vi "波形图.vi"() -> ()   [LabVIEW 2026]
doc: "波形图界面 - 测控软件 多链路实时波形展示。仅前面板布局演示，无程序逻辑。来源：波形图.html 主界面。"
panel:
  out "运行时长":string="运行时长: 00:00:00"
  out "通道":string="通道: 16"
  out "视图":string="视图: 0.0 - 30.0 s"
  out "窗口":string="窗口: 30.0 s"
  out "采样率":string="采样率: 100 Hz / 10 Hz"
  out "链路":string="链路: 4/4 在线"
  out "?":string="滚轮:缩放时间轴 · 左键框选放大 · 右键平移 · 双击复位"
  out "?":string="Δ值 --"
  out "?":string="Δt --"
  out "?":string="C2 --"
  out "?":string="C1 --"
  out "?":string="测量游标未放置 (0/2)"
  out "?":bool
  out "ARINC429 链路":bool=TRUE
  out "CAN 链路":bool=TRUE
  out "OPC 链路":bool=TRUE
  out "TCP 链路":bool=TRUE
  out "可见通道":i32=16
  out "总通道数":i32=23
  out "绘制帧率":string="60 fps"
  out "重绘周期":string="50 ms"
  out "?":string[](array[string])=["TCP(100 Hz · 10 通道): 转速(rpm) 24800", "TCP: 扭矩(N·m) 745", "TCP: 排气温度(℃) 662", "TCP: 滑油压力(kPa) 348", "TCP: 燃油流量(kg/h) 1240", "TCP: 起动信号 ON", "OPC(10 Hz · 5 通道): 28V母线电压(V) 28.10", "OPC: 28V母线电流(A) 12.40", "CAN(50 Hz · 4 通道): 发电机频率(Hz) 400", "ARINC429(20 Hz · 4 通道): 气压高度(m) 3200", "ARINC429: 马赫数 0.42"]
  out "?":waveform(dbl)(graph)
  out "?":string[](array[string])=["● 下位机 TCP | 192.168.1.101:8000 | PXIE-8840 环形缓冲 | 100 Hz | 10 通道", "● PLC OPC | opc.tcp://192.168.1.50:4840 | 西门子 S7-1500 OPC UA | 10 Hz | 5 通道", "● CAN 总线 | CAN1 · 500 kbps | PCIe-CAN-2 标准帧 | 50 Hz | 4 通道", "● ARINC429 | 429A/L0B1-L0B4 | PXIe-429-4 4发4收 | 20 Hz | 4 通道"]
  in  "通道过滤":i32(ring) items=["全部链路", "仅 TCP", "仅 OPC", "仅 CAN", "仅 ARINC429"]
  in  "Y轴模式":i32(ring) items=["百分比", "物理量程"]
  in  "窗口选择":i32(ring)=30 items=["5 s"=5, "10 s"=10, "15 s"=15, "30 s"=30, "60 s"=60, "120 s"=120]
  in  "清空缓冲":bool
  in  "导出图片":bool
  in  "清除游标":bool
  in  "放置游标":bool
  in  "复位视图":bool
  in  "暂停刷新":bool
  in  "滚动窗口":bool
  out "?":string="--:--:--"
  out "?":string="链路: 4/4 在线"
  out "?":string="● 波形图 | 测控软件 · 多链路实时波形展示"
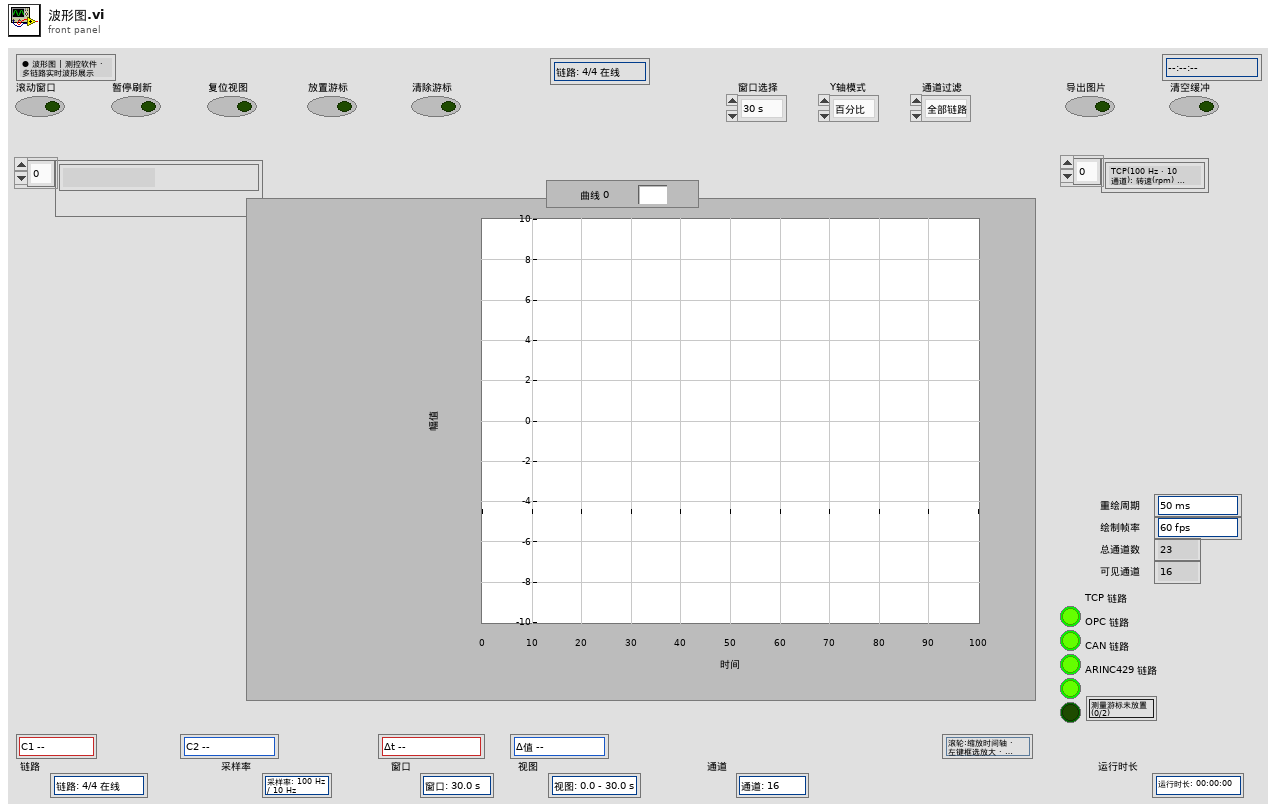
[diagram p1: front panel]
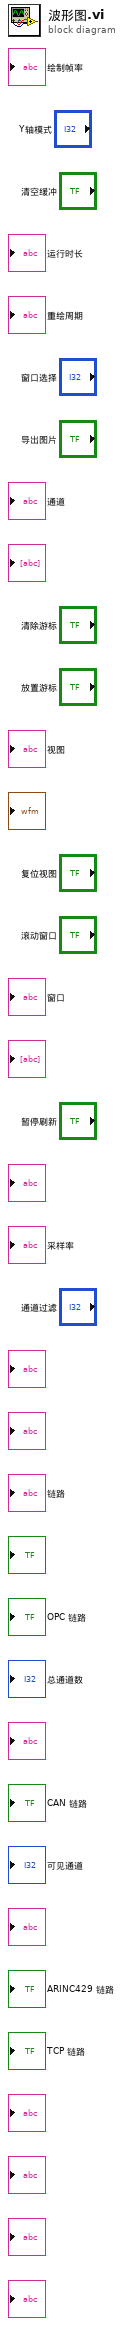
[diagram p0: block diagram]
diagram:
